vi "OwnOop20261013_ParentInfoV3.vi"() -> ()   [LabVIEW 2024]
panel:
  out "error out":errorcluster caption="错误输出"
  out "Parent Path":path
  out "Parent Name":string
  in  "Class Path":path
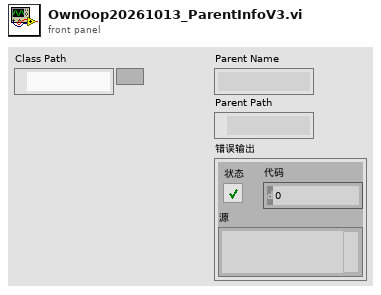
[diagram p1: front panel]
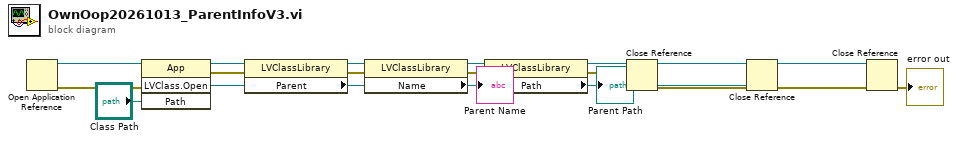
[diagram p0: block diagram]
diagram:
  n1 = Open Application Reference() -> (0:w12:errorcluster, 3:w14:refnum<vi>)  [unwired: 4 in]
  n2 = invoke class="App" method="LVClass.Open"(reference=w14, error in=w12, "Path"="Class Path") -> (error out=w10:errorcluster, "LVClass.Open"=w11:refnum<vi>)  [unwired: 1 in, 2 out]
  n3 = property class="LVClassLibrary"(reference=w11, error in=w10) -> (error out=w8:errorcluster, "Parent"=w9:refnum<vi>)  [unwired: 1 out]
  n4 = property class="LVClassLibrary"(reference=w9, error in=w8) -> (error out=w6:errorcluster, "Name"=→"Parent Name":string)  [unwired: 1 out]
  n5 = property class="LVClassLibrary"(reference=w9, error in=w6) -> (error out=w4:errorcluster, "Path"=→"Parent Path":path)  [unwired: 1 out]
  n6 = Close Reference(reference=w9, error in (no error)=w4) -> (error out=w3:errorcluster)
  n7 = Close Reference(reference=w11, error in (no error)=w3) -> (error out=w2:errorcluster)
  n8 = Close Reference(reference=w14, error in (no error)=w2) -> (error out=→"error out":errorcluster)
